vi "DSS-Tests-flatten_dbl_pair.vi"(11 "pair":cluster{"a":dbl[], "b":dbl[]}) -> (3 "flat":dbl[](array[numeric]))   [LabVIEW 2020, in "DSS-Tests.lvlib"]
doc: "Flattens a cluster of two 1D DBL arrays into one 1D DBL array: for each array in cluster order, the length followed by the elements."
uses:
  DSS-Tests.lvlib
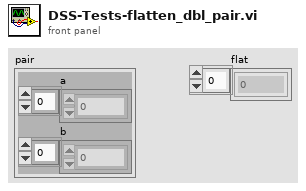
[diagram p1: front panel]
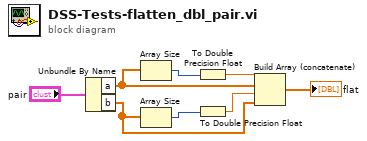
[diagram p0: block diagram]
diagram:
  n1 = Unbundle By Name("pair") -> ("a"=w2:dbl[], "b"=w3:dbl[])
  n2 = Array Size(array=w2) -> (size(s)=w4:i32)
  n3 = Array Size(array=w3) -> (size(s)=w6:i32)
  n4 = To Double Precision Float(number=w4) -> (double precision float=w5:dbl)
  n5 = To Double Precision Float(number=w6) -> (double precision float=w7:dbl)
  n6 = Build Array (concatenate)(w5, w2, w7, w3) -> (→"flat":dbl[])
